vi "test Quadrature.vi"(8 "error in (no error)":errorcluster, 11 "TestCase in":refnum<class "Scan Engine Specialty Digital System Tests.lvclass">) -> (0 "error out":errorcluster, 3 "TestCase out":refnum<class "Scan Engine Specialty Digital System Tests.lvclass">)   [LabVIEW 2020, in "Scan Engine Specialty Digital System Tests.lvclass"]
uses:
  Scan Engine Specialty Digital System Tests.lvclass
  C:/Program Files (x86)/National Instruments/LabVIEW 2020/vi.lib/NI/VeriStand Custom Device Testing Tools/VeriStandTestCase/VeriStandTestCase.lvclass
  <vilib>/addons/_JKI Toolkits/VI Tester/TestCase.llb/TestCase.lvclass
  <vilib>/NI/VeriStand Custom Device Testing Tools/VeriStandTestUtilities/VeriStandTestUtilities.lvlib
  C:/Program Files (x86)/National Instruments/LabVIEW 2020/vi.lib/addons/_JKI Toolkits/VI Tester/TestCase.llb/TestCase.lvclass
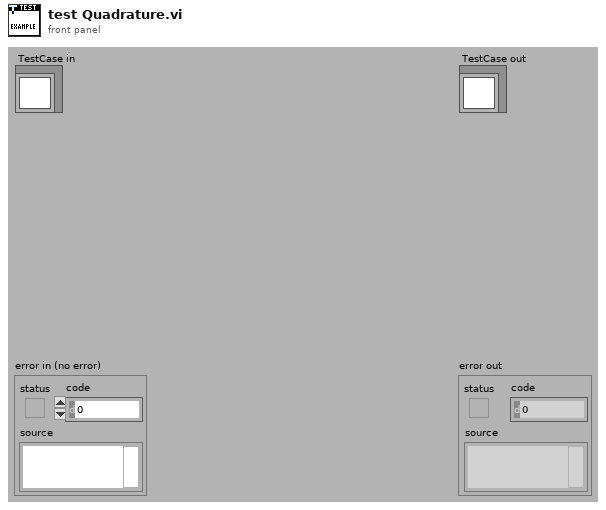
[diagram p1: front panel]
types:
  T1 = typedef "NI_VS Workspace ExecutionAPI.lvlib/WorkspaceAPI.ctl" = refnum<k24>
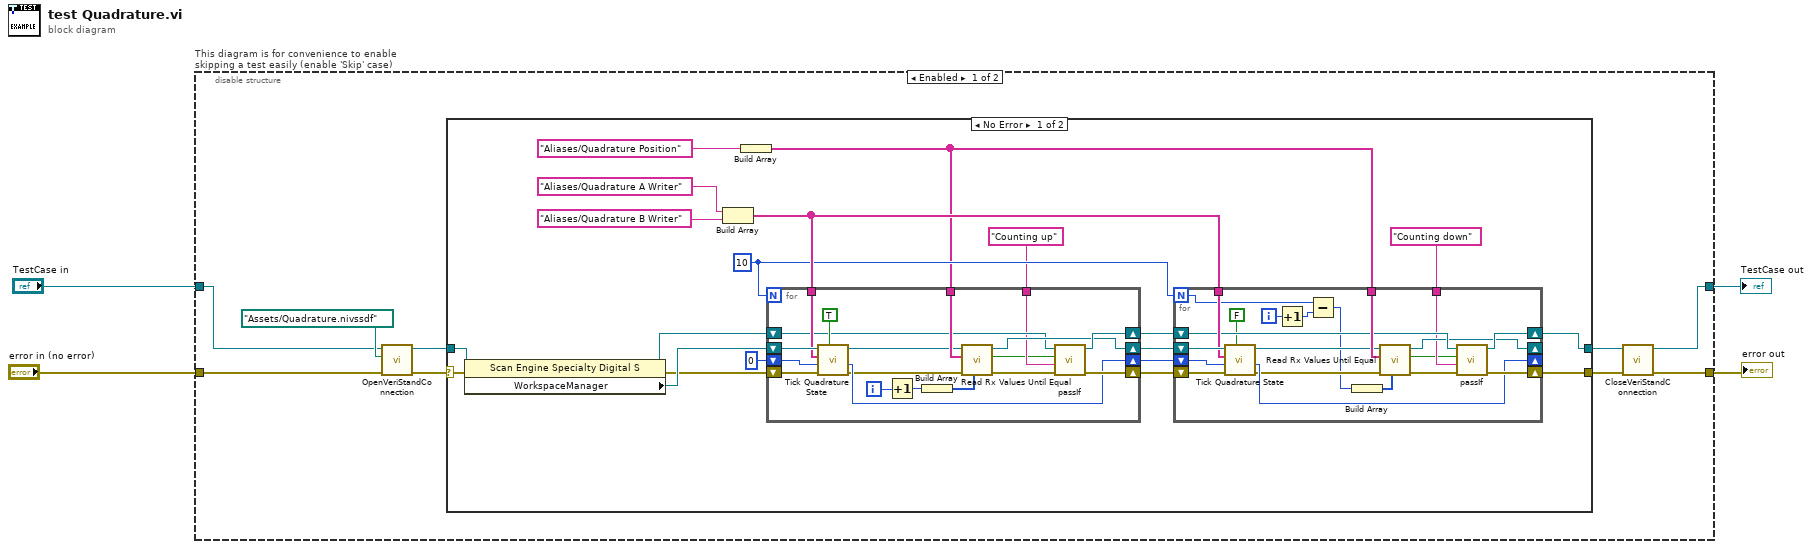
[diagram p0: block diagram]
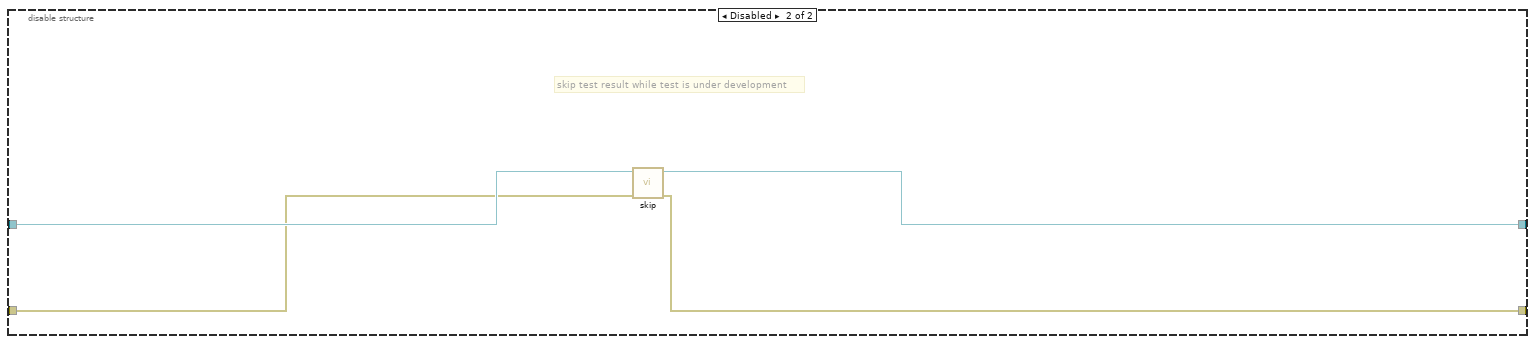
[diagram p3: hidden frame]
diagram:
  n1 = disable-structure "This diagram is for convenience to enable skipping a test easily (enable 'Skip' case)" shown="Enabled" {
    disable-tunnel: "TestCase in" -> [w9 w79]
    disable-tunnel: [w6 w77] -> w1
    disable-tunnel: [w7 w78] -> w3
    disable-tunnel: "error in (no error)" -> [w11 w76]
    frame Enabled {
      n2 = call-dynamic "OpenVeriStandConnection.vi"("error in (no error)"=w11, "System Definition File"=path "Assets/Quadrature.nivssdf", "VeriStand Test Case in"=w9) -> ("error out"=w12:errorcluster, "VeriStand Test Case out"=w10:refnum<class "Scan Engine Specialty Digital System Tests.lvclass">)  [unwired: 6 in, 1 out]
      n3 = case shown="No Error" w12 {
        selector: w12 -> [w33 w75]
        tunnel: [w18 w75] -> w8
        tunnel: [w17 w74] -> w5
        tunnel: w10 -> [w32 w74]
        frame No Error {
          w21 = 10
          n4 = property class="Scan Engine Specialty Digital S"(reference=w32, error in=w33) -> (reference out=w27:refnum<class "Scan Engine Specialty Digital System Tests.lvclass">, error out=w30:errorcluster, "WorkspaceManager"=w31:T1)
          n5 = Build Array("Aliases/Quadrature A Writer" ("Channel"), "Aliases/Quadrature B Writer" ("Channel")) -> (w25:string[])
          n6 = Build Array("Aliases/Quadrature Position" ("Channel")) -> (w14:string[])
          n7 = for {
            N: w21 -> [_]
            tunnel: w14 -> [w73]
            tunnel: w25 -> [w66]
            shift-right: [w71] -> w22
            shift-left: w30 -> [w67]
            shift-right: [w70] -> w23
            shift-left: w27 -> [w60]
            shift-right: [w64] -> w20
            shift-left: 0 ("New State") -> [w65]
            shift-right: [w63] -> w19
            shift-left: w31 -> [w68]
            tunnel: "Counting up" ("Channel") -> [w59]
            i -> [w61]
            n8 = call "Tick Quadrature State.vi"("Forward? (T)"=TRUE, "error in (no error)"=w67, "Current State"=w65, "Channels"=w66, "WorkspaceManager in"=w68) -> ("error out"=w58:errorcluster, "New State"=w64:i32, "WorkspaceManager out"=w69:T1)  [unwired: 4 in]
            n9 = Increment(x=w61) -> (x+1=w57:i32)
            n10 = Build Array(w57) -> (w56:i32[])
            n11 = call <vilib>:"Read Rx Values Until Equal.vi"("expected values"=w56, "error in"=w58, "Rx aliases"=w73, "workspace manager in"=w69) -> ("error out"=w72:errorcluster, "values equal expected"=w55:bool, "workspace manager out"=w63:T1)  [unwired: 5 in]
            n12 = call-dynamic "passIf.vi"("error in (no error)"=w72, "message (\"\")"=w59, "pass"=w55, "TestCase in"=w60) -> ("error out"=w71:errorcluster, "TestCase out"=w70:refnum<class "Scan Engine Specialty Digital System Tests.lvclass">)  [unwired: 6 in]
          }
          n13 = for {
            N: w21 -> [w41]
            tunnel: w14 -> [w54]
            tunnel: w25 -> [w47]
            shift-right: [w52] -> w18
            shift-left: w22 -> [w48]
            shift-right: [w51] -> w17
            shift-left: w23 -> [w46]
            shift-right: [w44] -> _
            shift-left: w20 -> [w45]
            shift-right: [w43] -> _
            shift-left: w19 -> [w49]
            tunnel: "Counting down" ("Channel") -> [w38]
            i -> [w40]
            n14 = call "Tick Quadrature State.vi"("Forward? (T)"=FALSE, "error in (no error)"=w48, "Current State"=w45, "Channels"=w47, "WorkspaceManager in"=w49) -> ("error out"=w37:errorcluster, "New State"=w44:i32, "WorkspaceManager out"=w50:T1)  [unwired: 4 in]
            n15 = Increment(x=w40) -> (x+1=w39:i32)
            n16 = Subtract(x=w41, y=w39) -> (x-y=w36:i32)
            n17 = Build Array(w36) -> (w35:i32[])
            n18 = call <vilib>:"Read Rx Values Until Equal.vi"("expected values"=w35, "error in"=w37, "Rx aliases"=w54, "workspace manager in"=w50) -> ("error out"=w53:errorcluster, "values equal expected"=w34:bool, "workspace manager out"=w43:T1)  [unwired: 5 in]
            n19 = call-dynamic "passIf.vi"("error in (no error)"=w53, "message (\"\")"=w38, "pass"=w34, "TestCase in"=w46) -> ("error out"=w52:errorcluster, "TestCase out"=w51:refnum<class "Scan Engine Specialty Digital System Tests.lvclass">)  [unwired: 6 in]
          }
        }
        frame Error {
        }
      }
      n20 = call-dynamic "CloseVeriStandConnection.vi"("error in (no error)"=w8, "VeriStand Test Case in"=w5) -> ("error out"=w7:errorcluster, "VeriStand Test Case out"=w6:refnum<class "Scan Engine Specialty Digital System Tests.lvclass">)  [unwired: 8 in]
    }
    frame Disabled {
      # "skip test result while test is under development"
      n21 = call <vilib>:"skip.vi"("error in (no error)"=w76, "TestCase in"=w79) -> ("error out"=w78:errorcluster, "TestCase out"=w77:refnum<class "Scan Engine Specialty Digital System Tests.lvclass">)  [unwired: 8 in]
    }
  }
  "error out" <- w3
  "TestCase out" <- w1
